vi "Set RIO INI Key.vi"(8 "error in (no error)":errorcluster, 11 "Section Ref in":T1 format="%.0x") -> (0 "error out":errorcluster, 3 "Section Ref out":T1 format="%.0x")   [LabVIEW 2020, in "FPGA Addon Engine.lvlib"]
uses:
  FPGA Addon Engine.lvlib
  <vilib>/NI VeriStand/Custom Device API/Custom Device Item Ref.ctl
  <vilib>/Utility/config.llb/Write Key (I32).vi
  <vilib>/Utility/config.llb/NI_LVConfig.lvlib
  <vilib>/NI VeriStand/Custom Device API/Custom Device API.lvlib
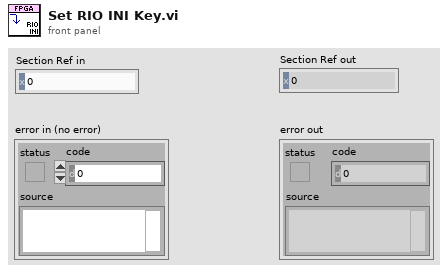
[diagram p1: front panel]
types:
  T1 = typedef "Custom Device API.lvlib/Custom Device Item Ref.ctl" = u64
  T2 = typedef "Custom Device API.lvlib/Custom Device Target Type.ctl" = enum16{"PharLap", "VxWorks", "Windows", "Linux_32_ARM", "Linux_x64"}
  T3 = typedef "NI_LVConfig.lvlib/Config Data RefNum.ctl" = refnum<k1>
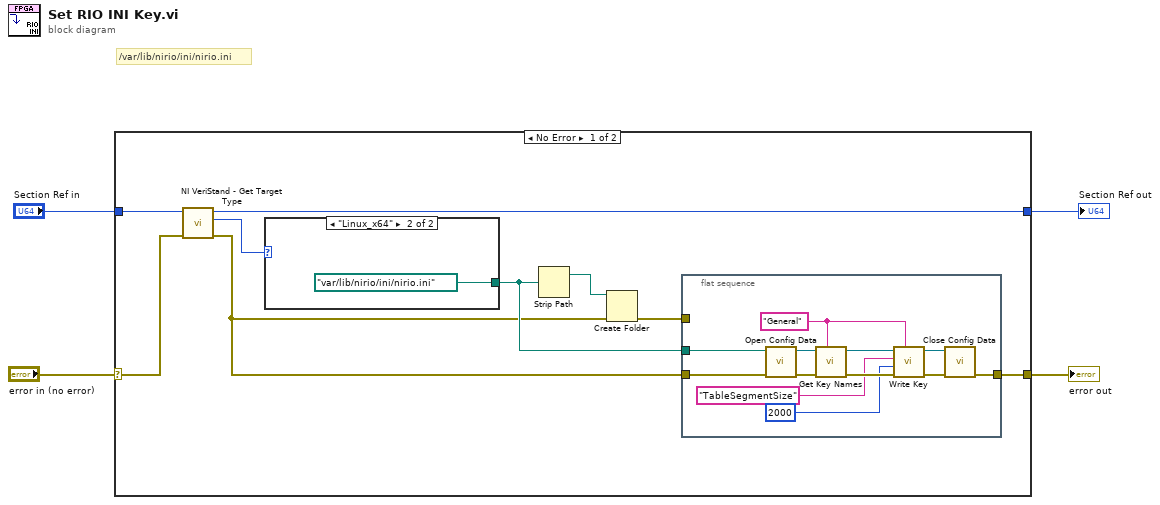
[diagram p0: block diagram]
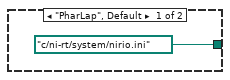
[diagram p2: hidden frame]
diagram:
  # "/var/lib/nirio/ini/nirio.ini"
  n1 = case shown="No Error" "error in (no error)" {
    selector: "error in (no error)" -> [w5 w28]
    tunnel: [w13 w28] -> w4
    tunnel: "Section Ref in" -> [w10 w29]
    tunnel: [w6 w29] -> w2
    frame No Error {
      n2 = call <vilib>:"NI VeriStand - Get Target Type.vi"("error in (no error)"=w5, "Item Ref in"=w10) -> ("error out"=w7:errorcluster, "Target Type"=w9:T2, "Item Ref out"=w6:T1)  [unwired: 7 in]
      n3 = case shown="\"Linux_x64\"" w9 {
        tunnel: [path "c:/ni-rt/system/nirio.ini" ("configuration file path") path "/var/lib/nirio/ini/nirio.ini" ("configuration file path")] -> w8
        frame "PharLap", Default {
        }
        frame "Linux_x64" {
        }
      }
      n4 = Strip Path(path=w8) -> (stripped path=w12:path)  [unwired: 1 out]
      n5 = Create Folder(path (use dialog)=w12, error in=w7) -> (error out=w11:errorcluster)  [unwired: 1 in, 2 out]
      n6 = flat-sequence {
        tunnel: [w18] -> w13
        tunnel: w8 -> [w17]
        tunnel: w7 -> [w16]
        tunnel: w11 -> [_]
        frame #0 {
          w24 = "General" ("section")
          n7 = call <vilib>:"Open Config Data.vi"("error in (no error)"=w16, "configuration file path"=w17) -> ("error out"=w27:errorcluster, "refnum"=w26:T3)  [unwired: 7 in, 1 out]
          n8 = call <vilib>:"Get Key Names.vi"("section"=w24, "error in (no error)"=w27, "refnum"=w26) -> ("error out"=w23:errorcluster, "refnum out"=w25:T3)  [unwired: 5 in, 2 out]
          n9 = call-poly <vilib>:"Write Key.vi"("section"=w24, "error in (no error)"=w23, "value"=2000, "key"="TableSegmentSize", "refnum"=w25) -> ("error out"=w19:errorcluster, "refnum out"=w22:T3)  [unwired: 4 in, 1 out]
          n10 = call <vilib>:"Close Config Data.vi"("error in (no error)"=w19, "refnum"=w22) -> ("error out"=w18:errorcluster)  [unwired: 8 in, 1 out]
        }
      }
    }
    frame Error {
    }
  }
  "error out" <- w4
  "Section Ref out" <- w2
